vi "SUP_Camera_Observe_U8_UNCOMPILED.vi"(4 "valeur de l'horloge en ms 3":u32, 5 "valeur de l'horloge en ms 2":u32, 6 "valeur de l'horloge en ms":u32, 7 "temps actuel 3":timestamp, 8 "temps actuel 2":timestamp, 9 "temps actuel":timestamp, 10 "error in (no error)":errorcluster, 11 "Image":T1) -> (0 "error out":errorcluster, 1 "error in (no error) 3":errorcluster, 2 "error in (no error) 2":errorcluster, 3 "Image 2":T1)   [LabVIEW 2012]
uses:
  <vilib>/vision/Image Controls.llb/IMAQ Image.ctl
panel:
  out "Image Pixels (I16)":i16[][](array[numeric])
  out "Image Pixels (U8)":u8[][](array[numeric])
  out "Image Pixels (Float)":sgl[][](array[numeric]) format="%.2f"
  out "Image Pixels (U16)":u16[][](array[numeric])
  in  "Optional Rectangle":i32[](array[numeric])
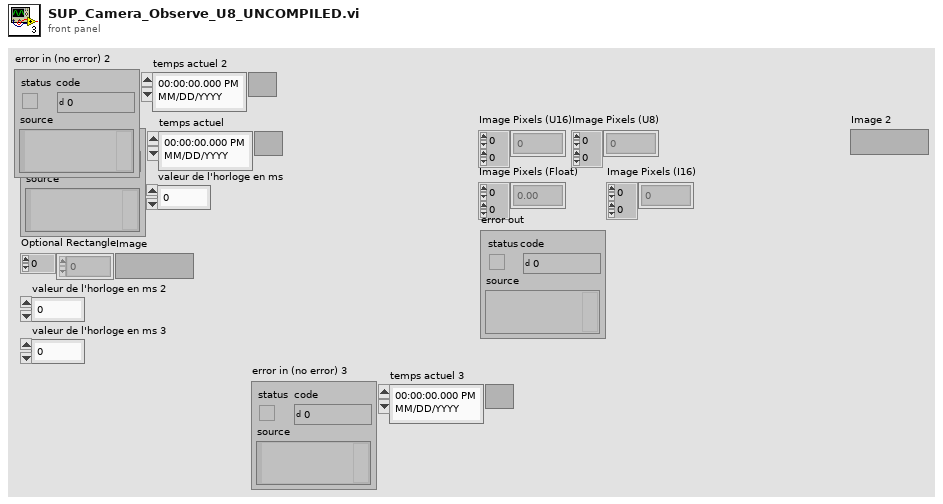
[diagram p1: front panel]
types:
  T1 = typedef "IMAQ Image.ctl" = refnum<image>
  T2 = cluster{"source":string, u16, "temps actuel":timestamp, "temps actuel 2":timestamp, "temps actuel 3":timestamp, "valeur de l'horloge en ms 3":u32, "valeur de l'horloge en ms 3":u32}
  T3 = cluster{u32, "valeur de l'horloge en ms 3":u32, "Image Pixels (U8)":u8[][]}
  T4 = cluster{cluster{"source":string, u16, "temps actuel":timestamp, "temps actuel 2":timestamp, "temps actuel 3":timestamp, "valeur de l'horloge en ms 3":u32, "valeur de l'horloge en ms 3":u32}, cluster{u32, "valeur de l'horloge en ms 3":u32, "Image Pixels (U8)":u8[][]}}
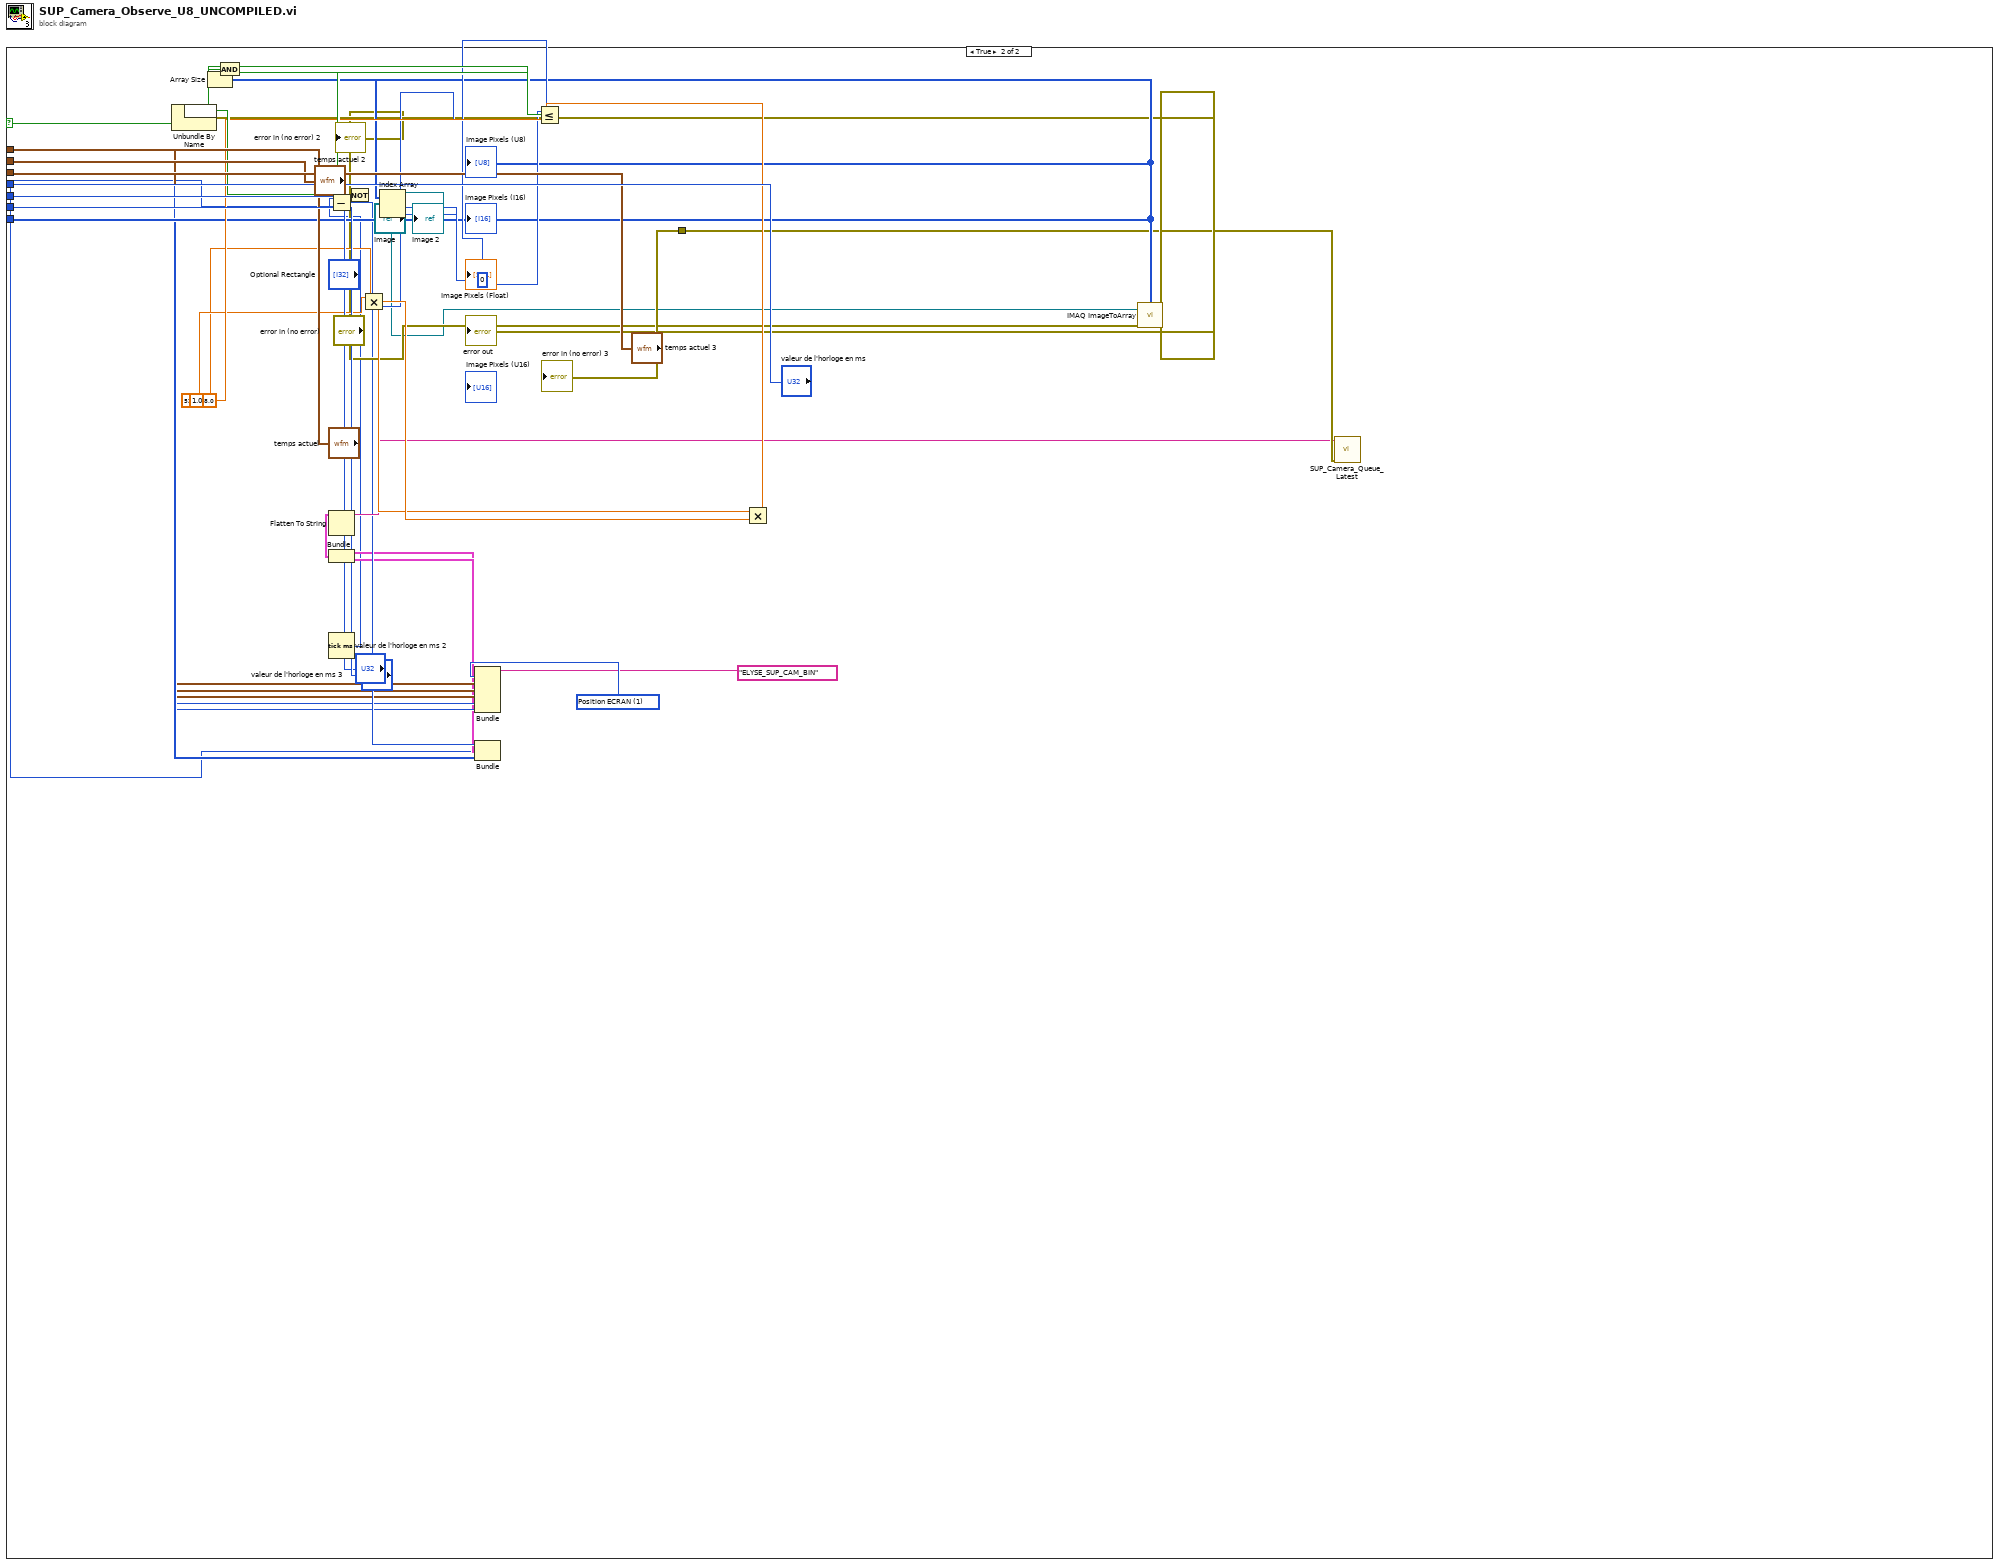
[diagram p0: block diagram]
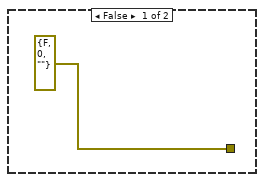
[diagram p2: hidden frame]
diagram:
  n1 = call "IMAQ ImageToArray"("error in (no error)"="error in (no error)", "Image"="Image") -> ("error out"=w3:errorcluster, "Image Pixels (U8)"=w4:u8[][])  [unwired: 2 in, 3 out]
  "error out" <- w3
  "Image Pixels (U8)" <- w4
  n2 = Unbundle By Name(w3) -> (w22:bool)
  n3 = Array Size(array=w4) -> (size(s)=w5:i32[])
  n4 = Not(x=w22) -> (.not. x?=w24:bool)
  n5 = Index Array(array=w5, index #1=0 ("Motor position"), index #2=1 ("Motor position")) -> (element #1=w9:i32, element #2=w12:i32)
  n6 = Multiply(x=1.0 ("Échelle des X.Gamme : minimum"), y=w9) -> (x*y=w14:dbl)
  n7 = Multiply(x=1.0 ("Échelle des X.Gamme : minimum"), y=w12) -> (x*y=w15:dbl)
  n8 = Less Or Equal?(x=1 ("Motor position"), y=w9) -> (x <= y?=w18:bool)
  n9 = Less Or Equal?(x=1 ("Motor position"), y=w12) -> (x <= y?=w19:bool)
  n10 = And(x=w18, y=w19) -> (x .and. y?=w20:bool)
  n11 = Multiply(x=w14, y=w15) -> (x*y=w16:dbl)
  n12 = Less Or Equal?(x=w16, y=524288.0 ("Échelle des X.Gamme : minimum")) -> (x <= y?=w21:bool)
  n13 = And(x=w20, y=w21) -> (x .and. y?=w23:bool)
  n14 = And(x=w23, y=w24) -> (x .and. y?=w25:bool)
  n15 = case shown="True" w25 {
    tunnel: "temps actuel" -> [_ w41]
    tunnel: "temps actuel 2" -> [_ w42]
    tunnel: "temps actuel 3" -> [_ w43]
    tunnel: "valeur de l'horloge en ms" -> [_ w44]
    tunnel: "valeur de l'horloge en ms 2" -> [_ w45]
    tunnel: "valeur de l'horloge en ms 3" -> [_ w35]
    tunnel: w4 -> [_ w47]
    tunnel: [errorcluster {"status"=FALSE, "code"=0, "source"=""} ("error IO") w49] -> w32
    frame False {
    }
    frame True {
      w40 = u16 1 items=["Position FAISCEAU", "Position ECRAN", "Position CERENKOV"] ("Position diagnostique T1")
      n16 = Tick Count (ms)() -> (millisecond timer value=w34:u32)
      n17 = Subtract(x=w34, y=w35) -> (x-y=w46:u32)
      n18 = Bundle("source"="ELYSE_SUP_CAM_BIN" ("camera_magic"), w40, "temps actuel"=w41, "temps actuel 2"=w42, "temps actuel 3"=w43, "valeur de l'horloge en ms 3"=w44, "valeur de l'horloge en ms 3"=w45) -> (w36:T2)  [unwired: 1 in]
      n19 = Bundle(w46, "valeur de l'horloge en ms 3"=w35, "Image Pixels (U8)"=w47) -> (w37:T3)  [unwired: 1 in]
      n20 = Bundle(w36, w37) -> (w38:T4)  [unwired: 1 in]
      n21 = Flatten To String(anything=w38) -> (data string=w48:string)  [unwired: 3 in, 2 out]
      n22 = call "SUP_Camera_Queue_Latest.vi"("packet"=w48) -> ("telemetry error"=w49:errorcluster)  [unwired: 9 in, 1 out]
    }
  }
  "error in (no error) 3" <- w32
  "error in (no error) 2" <- "error in (no error)"
  "Image 2" <- "Image"
